vi "Element Init.vi"(7 "VolatusAPI":refnum<class "VolatusAPI.lvclass">, 8 "error in (no error)":errorcluster, 10 "JSON":string, 11 "SystemConfigStatusIndicator in":refnum<class "SystemConfigStatusIndicator.lvclass">) -> (0 "error out":errorcluster, 3 "SystemConfigStatusIndicator out":refnum<class "SystemConfigStatusIndicator.lvclass">)   [LabVIEW 2020, in "VolatusGUIElements.lvlib" / "SystemConfigStatusIndicator.lvclass"]
uses:
  SystemConfigStatusIndicator.lvclass
  Volatus/VolatusAPI/VolatusAPI.lvclass
  JSON.ctl
  Volatus/Config Monitor Identity/Config Monitor Identity.lvclass
  C:/dev/lv20CE/relink/lv-volatus/Volatus/Identity/Identity.lvclass
  Volatus/System Config Status API/System Config Status API.lvclass
  C:/dev/lv20CE/relink/lv-promises/Promises/Value/Value.lvclass
  Volatus/VolatusAPI/VolatusAPI.lvclass/VolatusAPI.ctl
  SystemConfigStatusIndicator.lvclass/SystemConfigStatusIndicator.ctl
  0a9e5f5f-8607-4ac1-b9a2-f4ba17706565.vi
  <vilib>/JDP Science/JSONtext/JSON text to Variant.vi
  <vilib>/JDP Science/JSONtext/LVClass Serializer/JSONtext LVClass Serializer.lvclass
  VolatusConfig/Node/Node Config.lvclass
  lv-vecto/Vecto/Node Config/Node Config.lvclass
  Volatus/MessageQ/MessageQ.lvclass
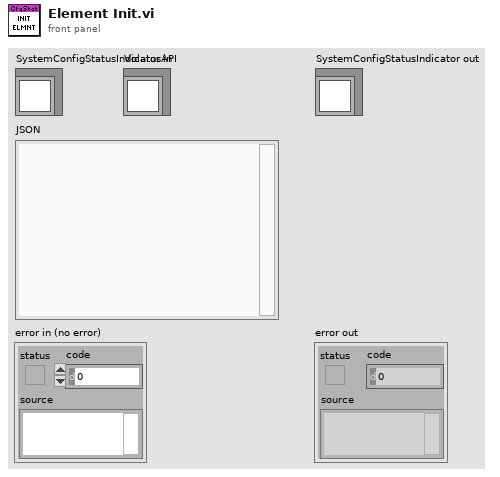
[diagram p1: front panel]
types:
  T1 = typedef "VolatusGUIElements.lvlib/SystemConfigStatusIndicator.lvclass/JSON.ctl" = cluster{"Exclude":string[], "Staleness":dbl}
  T2 = typedef "VectoConfig.lvlib/Node Info.ctl" = cluster{"System":string, "Cluster":string, "Name":string, "ID":u32, "Capabilities":string[]}
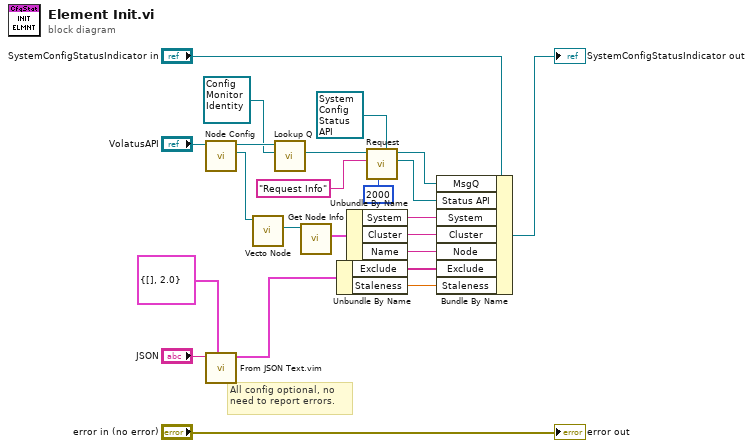
[diagram p0: block diagram]
diagram:
  # "All config optional, no need to report errors."
  n1 = call "Node Config.vi"("VolatusAPI in"="VolatusAPI") -> ("Node Config"=w18:refnum<class "Node Config.lvclass">, "VolatusAPI out"=w9:refnum<class "VolatusAPI.lvclass">)  [unwired: 9 in]
  n2 = call "From JSON Text.vim"("Data Type and Default Value"=T1 {"Exclude"=[], "Staleness"=2.0} ("JSON"), "JSON"="JSON") -> ("Data out"=w11:T1)  [unwired: 8 in, 1 out]
  n3 = call "Vecto Node.vi"("Node in"=w18) -> ("Vecto Node"=w17:refnum<class "Node Config.lvclass">)  [unwired: 8 in, 2 out]
  n4 = call "Lookup Q.vi"("Identity"=refnum<class "Config Monitor Identity.lvclass"> refnum ("Volatus:Config Monitor Identity.lvclass"), "VolatusAPI in"=w9) -> ("MessageQ"=w5:refnum<class "MessageQ.lvclass">)  [unwired: 7 in, 2 out]
  n5 = call "Get Node Info.vi"("Node Config in"=w17) -> ("Info"=w16:T2)  [unwired: 8 in, 2 out]
  n6 = Unbundle By Name(w11) -> ("Exclude"=w10:string[], "Staleness"=w7:dbl)
  n7 = Unbundle By Name(w16) -> ("System"=w14:string, "Cluster"=w13:string, "Name"=w12:string)
  n8 = call "Request.vi"("Response Value Type"=refnum<class "System Config Status API.lvclass"> refnum ("Status API"), "Timeout ms (1000)"=2000, "ID"="Request Info", "MessageQ in"=w5) -> ("Response"=w4:refnum<class "System Config Status API.lvclass">, "MessageQ out"=w1:refnum<class "MessageQ.lvclass">)  [unwired: 5 in, 1 out]
  n9 = Bundle By Name(cluster="SystemConfigStatusIndicator in", "MsgQ"=w1, "Status API"=w4, "System"=w14, "Cluster"=w13, "Node"=w12, "Exclude"=w10, "Staleness"=w7) -> (→"SystemConfigStatusIndicator out":refnum<class "SystemConfigStatusIndicator.lvclass">)
  "error out" <- "error in (no error)"
